vi "libssh2_sftp_get_channel.vi"(8 "error in (no error)":errorcluster, 11 "sftp":T2) -> (0 "error out":errorcluster, 3 "channel":T1)   [LabVIEW 2017, in "libssh2.lvlib"]
doc: "Get the channel associated with an SFTP session."
uses:
  libssh2.lvlib
  SFTP Refnum.ctl
  Channel Refnum.ctl
  Acquire Session.vi
  Release Session.vi
  Not An SFTP Refnum.vi
  <vilib>/Utility/error.llb/Error Cluster From Error Code.vi
  Global Settings.vi
  Read Session Refnum.vi
  <vilib>/Utility/semaphor.llb/Acquire Semaphore.vi
  <vilib>/Utility/semaphor.llb/Release Semaphore.vi
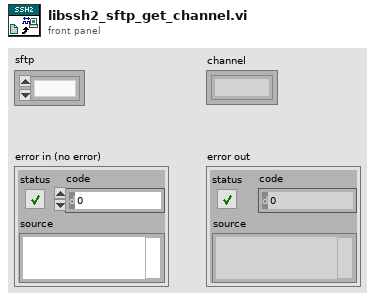
[diagram p1: front panel]
types:
  T1 = typedef "libssh2.lvlib/Channel Refnum.ctl" = refnum<k1>
  T2 = typedef "libssh2.lvlib/SFTP Refnum.ctl" = refnum<k1>
  T3 = typedef "libssh2.lvlib/Session Refnum.ctl" = refnum<k1>
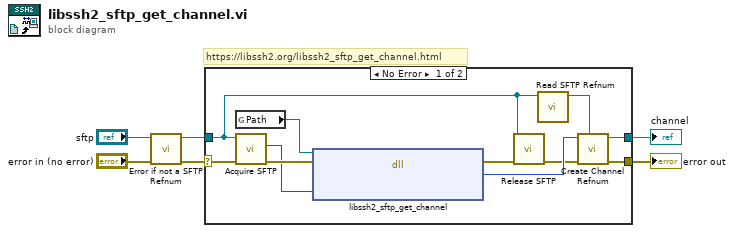
[diagram p0: block diagram]
diagram:
  # "https://libssh2.org/libssh2_sftp_get_channel.html"
  n1 = call "Error if not a SFTP Refnum.vi"("error in (no error)"="error in (no error)", "sftp"="sftp") -> ("error out"=w5:errorcluster, "sftp out"=w4:T2)  [unwired: 8 in]
  n2 = case shown="No Error" w5 {
    selector: w5 -> [w16 w18]
    tunnel: w4 -> [w8 _]
    tunnel: [w12 w18] -> w3
    tunnel: [w10 _] -> w1
    frame No Error {
      n3 = global read "Global Settings.vi" "Path"() -> (w17:path)
      n4 = call "Acquire SFTP.vi"("error in (no error)"=w16, "sftp"=w8) -> ("error out"=w15:errorcluster, "LIBSSH2_SFTP*"=w14:u64)  [unwired: 8 in]
      n5 = dll-call lib="?" fn="libssh2_sftp_get_channel"(path in=w17, error in=w15, "sftp"=w14) -> (error out=w13:errorcluster, "return value"=w11:u64)  [unwired: 2 in, 1 out]
      n6 = call "Release SFTP.vi"("error in (no error)"=w13, "sftp"=w8) -> ("error out"=w9:errorcluster)  [unwired: 9 in]
      n7 = call "Read SFTP Refnum.vi"("sftp"=w8) -> ("session"=w7:T3)  [unwired: 8 in, 2 out]
      n8 = call "Create Channel Refnum.vi"("session"=w7, "error in (no error)"=w9, "LIBSSH2_CHANNEL*"=w11) -> ("error out"=w12:errorcluster, "channel"=w10:T1)  [unwired: 7 in]
    }
    frame Error {
    }
  }
  "error out" <- w3
  "channel" <- w1
